vi "XPN Get Acquisition Time.vi"(8 "error in (no error)":errorcluster, 11 "timeMs":i32) -> (0 "error out":errorcluster, 2 "function return":i32, 3 "timeMs out":i32)   [LabVIEW 2025, in "xPanelWrapper.lvlib"]
doc: "XPN_API int XPN_GetAcquisitionTime(int* timeMs);"
uses:
  xPanelWrapper.lvlib
  xPanelWrapper.dll
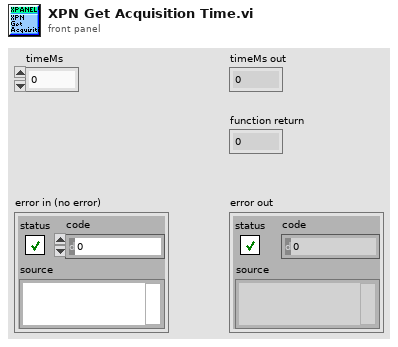
[diagram p1: front panel]
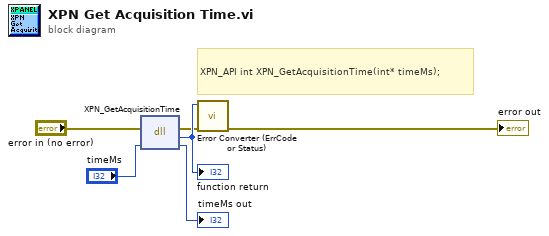
[diagram p0: block diagram]
diagram:
  # "XPN_API int XPN_GetAcquisitionTime(int* timeMs);"
  n1 = dll-call lib="C:/Users/AriNutpam User/Documents/GitHub/The-Oracle/Image Acquisition/Child Classes/DTImager/xPanelWrapperLvLib/xPanelWrapper.*" fn="XPN_GetAcquisitionTime"(error in="error in (no error)", "timeMs"="timeMs") -> (error out=w2:errorcluster, w6:i32, "timeMs"=→"timeMs out":i32)  [unwired: 2 in, 1 out]
  "function return" <- w6
  n2 = call "Error Converter (ErrCode or Status).vi"("error in (no error)"=w2, "error code"=w6) -> ("error out"=→"error out":errorcluster)  [unwired: 9 in]
